vi "Send Command.vi"(7 "VolatusAPI":refnum<class "VolatusAPI.lvclass">, 8 "error in (no error)":errorcluster, 10 "Value":bool, 11 "2WayValve in":refnum<class "2WayValveV.lvclass">) -> (0 "error out":errorcluster, 3 "2WayValve out":refnum<class "2WayValveV.lvclass">)   [LabVIEW 2020, in "VolatusGUIElements.lvlib" / "2WayValveV.lvclass"]
uses:
  2WayValveV.lvclass
  C:/dev/lv20CE/relink/lv-volatus/VolatusGUI/GUI Element/GUI Element.lvclass
  Volatus/VolatusAPI/VolatusAPI.lvclass
  2WayValveV.lvclass/2WayValveV.ctl
  messages/CmdDigital/Class/Msg.lvclass/Msg.ctl
  Volatus/VolatusAPI/VolatusAPI.lvclass/VolatusAPI.ctl
  messages/CmdDigital/Class/Msg.lvclass
  C:/dev/lv20CE/relink/lv-protoc/LV-Proto/Message/Message.lvclass
  lv-vecto/Vecto/TCPMessageService/Send Message.vi
  <vilib>/Utility/error.llb/Error Cluster From Error Code.vi
  lv-protoc/LV-Proto/Message/Message.lvclass
  VolatusGUI/GUI Element/GUI Element.lvclass
  Volatus/Digital Command/Digital Command.lvclass
  C:/dev/lv20CE/relink/lv-volatus/VolatusGUIElements/2WayValveV/2WayValveV.lvclass
  C:/dev/lv20CE/relink/lv-volatus/VolatusGUI/OnValueChangeHandler/OnValueChangeHandler.lvclass
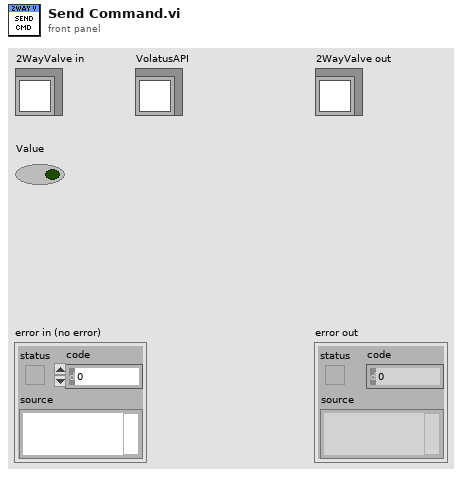
[diagram p1: front panel]
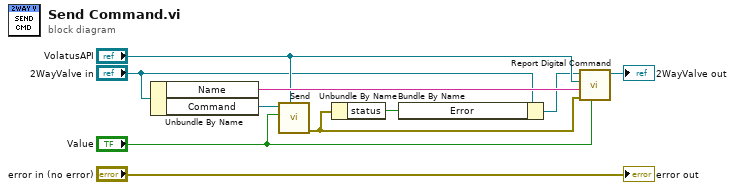
[diagram p0: block diagram]
diagram:
  n1 = Unbundle By Name("2WayValve in") -> ("Name"=w9:string, "Command"=w8:refnum<class "Digital Command.lvclass">)
  n2 = call "Send.vi"("VolatusAPI"="VolatusAPI", "Value"="Value", "Digital Command in"=w8) -> ("error out"=w5:errorcluster)  [unwired: 7 in, 1 out]
  n3 = Unbundle By Name(w5) -> ("status"=w3:bool)
  n4 = Bundle By Name(cluster="2WayValve in", "Error"=w3) -> (w2:refnum<class "2WayValveV.lvclass">)
  n5 = call "Report Digital Command.vi"("Value"="Value", "error in (no error)"=w5, "Name"=w9, "VolatusAPI in"="VolatusAPI", "GUI Element in"=w2) -> ("GUI Element out"=→"2WayValve out":refnum<class "2WayValveV.lvclass">)  [unwired: 5 in, 1 out]
  "error out" <- "error in (no error)"
